vi "FuncVI-FFT2D.vi"(5 "InstanceRef":T2, 9 "arg list":T1[](array[typedef]) {"num" format="%.2f"}) -> (0 "error out":bool, 3 "result":T1 {"num" format="%.2f"})   [LabVIEW 2021]
doc: "<B>FuncVI-FFT2D</B>\n\nThis VI is example of implementation of CalcExpress function (FuncVI). The function computes FFT on input 2D array.\n\n::: CalcExpress Toolkit :::\nCopyright (c) 2000-2026 Konstantin Shifershteyn. All rights reserved."
uses:
  vi.lib/addons/CalcExpress/cetypes.llb/CalcExpress Function Argument Info.ctl
  vi.lib/addons/CalcExpress/cetypes.llb/CalcExpress Instance RefNum.ctl
  <vilib>/Analysis/2dsp.llb/Real FFT.vi
  <vilib>/Analysis/2dsp.llb/Complex FFT.vi
  <vilib>/Analysis/NI_AALPro.lvlib
panel:
  in  "max arg num":i32=1
  in  "min arg num":i32=1
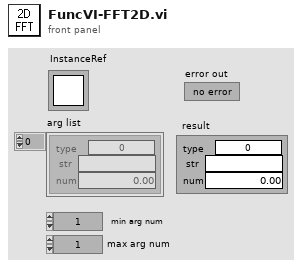
[diagram p1: front panel]
types:
  T1 = typedef "CalcExpress Function Argument Info.ctl" = cluster{"type":u32, "str":string, "num":dbl}
  T2 = typedef "CalcExpress Instance RefNum.ctl" = refnum<k1>
  T3 = enum32{"String", "DBL Number", "identifier", "1D Array of DBL", "2D Array of DBL", "CDB Number", "1D Array of CDB", "2D Array of CDB", "1D Array of String", "2D Array of String", "Unknown data type"}
  T4 = cluster{"index":i32, "data type":enum32{"String", "DBL Number", "identifier", "1D Array of DBL", "2D Array of DBL", "CDB Number", "1D Array of CDB", "2D Array of CDB", "1D Array of String", "2D Array of String", "Unknown data type"}, "default num":dbl, "default str":string}[]
  T5 = cluster{"data type":enum32{"String", "DBL Number", "identifier", "1D Array of DBL", "2D Array of DBL", "CDB Number", "1D Array of CDB", "2D Array of CDB", "1D Array of String", "2D Array of String", "Unknown data type"}, "data string":string, dbl}
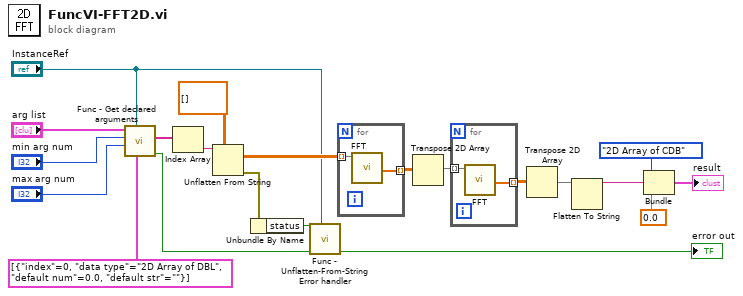
[diagram p0: block diagram]
diagram:
  n1 = call "Func - Get declared arguments.vi"("arg descriptors"=T4 [{"index"=0, "data type"=enum."2D Array of DBL", "default num"=0.0, "default str"=""}] ("args descriptors"), "InstanceRef"="InstanceRef", "max arg num"="max arg num", "min arg num"="min arg num", "arg list"="arg list") -> ("error out"=w5:bool, "str list"=w16:string[])  [unwired: 3 in, 2 out]
  n2 = Index Array(array=w16) -> (element=w15:string)  [unwired: 1 in]
  n3 = Unflatten From String(type=dbl[][] [], binary string=w15) -> (value=w13:dbl[][], error out=w1:errorcluster)  [unwired: 3 in, 1 out]
  n4 = Unbundle By Name(w1) -> ("status"=w3:bool)
  n5 = call "Func - Unflatten-From-String Error handler.vi"("InstanceRef"="InstanceRef", "error in"=w5, "Unflatten Error status"=w3) -> ("error out"=→"error out":bool)  [unwired: 6 in]
  n6 = for {
    tunnel: w13 -> [w23] mode=indexing
    tunnel: [w22] -> w12 mode=indexing
    n7 = call-poly <vilib>:"FFT.vi"("X"=w23) -> ("FFT {X}"=w22:cdb[])  [unwired: 9 in, 1 out]
  }
  n8 = Transpose 2D Array(2D array=w12) -> (transposed array=w9:cdb[][])
  n9 = for {
    tunnel: w9 -> [w25] mode=indexing
    tunnel: [w24] -> w10 mode=indexing
    n10 = call-poly <vilib>:"FFT.vi"("X"=w25) -> ("FFT {X}"=w24:cdb[])  [unwired: 9 in, 1 out]
  }
  n11 = Transpose 2D Array(2D array=w10) -> (transposed array=w8:cdb[][])
  n12 = Flatten To String(anything=w8) -> (data string=w11:string)  [unwired: 3 in, 2 out]
  n13 = Bundle("data type"=T3."2D Array of CDB", "data string"=w11, 0.0) -> (→"result":T5)  [unwired: 1 in]
